vi "Measurement Logic.vi"() -> ()   [LabVIEW 2021, in "Short-Circuit.lvlib"]
uses:
  Short-Circuit.lvlib
  <vilib>/Plug-In SDKs/Measurements/Measure Call Context/Measure Call Context.lvclass
  Measurement Configuration.ctl
  Measurement Results.ctl
  Controls/LED_SCT_Data.ctl
  <instrlib>/niDCPower/nidcpower.llb/niDCPower Source Mode.ctl
  <instrlib>/niDCPower/nidcpower.llb/niDCPower Wait For Event - Event.ctl
  <instrlib>/niSwitch/niSwitch.llb/niSwitch Relay Action.ctl
  <instrlib>/niDMM/nidmm.llb/niDMM Function.ctl
  <instrlib>/niDCPower/nidcpower.llb/niDCPower Output Function.ctl
  <instrlib>/niDCPower/nidcpower.llb/niDCPower Get Channel Name From String.vi
  <instrlib>/niDMM/nidmm.llb/niDMM Configure Measurement Digits.vi
  <instrlib>/niDCPower/nidcpower.llb/niDCPower Configure Digital Edge Source Trigger With Channels.vi
  <instrlib>/niDCPower/nidcpower.llb/niDCPower Configure Digital Edge Measure Trigger With Channels.vi
panel:
  out "measurement results":T1={"Status"="Empty", "Source voltages"=[0.0], "Load voltages"=[0.0], "Source Current"=[0.0], "Load Current"=[0.0]}
  in  "measurement configuration":T2={"DUT setup time"=0.5, "Source delay"=0.5, "Aperture time"=0.5, "Source resource name"="Lorem ipsum dolor sit", "Source sense"=64, "Source current limit"=2.0, "Source maximum power"=20.0, "Source Voltage (Vo)"=3.5, "Load resource name"="", "Load sense"=-64, "Load voltage limit range"=60.0, "Load Voltage Limit"=6.0, "Load Current Level (Io)"=0.1, "Switch resource name"="", "Switch - Load Relay Name"="", "Switch - DMM Relay Name"="", "Relay Topology"="Configured Topology", "DMM resource name"="", "DMM Current Range(A)"=3.0, "SC - Trigger Delay (sec)"=5.0, "SC - Hold Delay (sec)"=5.0, "Resolution in Digits"=6.5} {"Resolution in Digits" items=["3 1/2"=3.5, "4 1/2"=4.5, "5 1/2"=5.5, "6 1/2"=6.5, "7 1/2"=7.5]; "Load Current Level (Io)" format="%.3f"; "Source Voltage (Vo)" format="%.2f"; "Load sense" items=["Local"=1008, "Remote"=1009]; "Source sense" items=["Local"=1008, "Remote"=1009]; "Aperture time" format="%#_6p"; "Source delay" format="%#_6p"; "DUT setup time" format="%#_6p"}
  out "measure call context out":refnum<class "Measure Call Context.lvclass">
  in  "measure call context in":refnum<class "Measure Call Context.lvclass">
  out "error out":errorcluster
  in  "error in":errorcluster
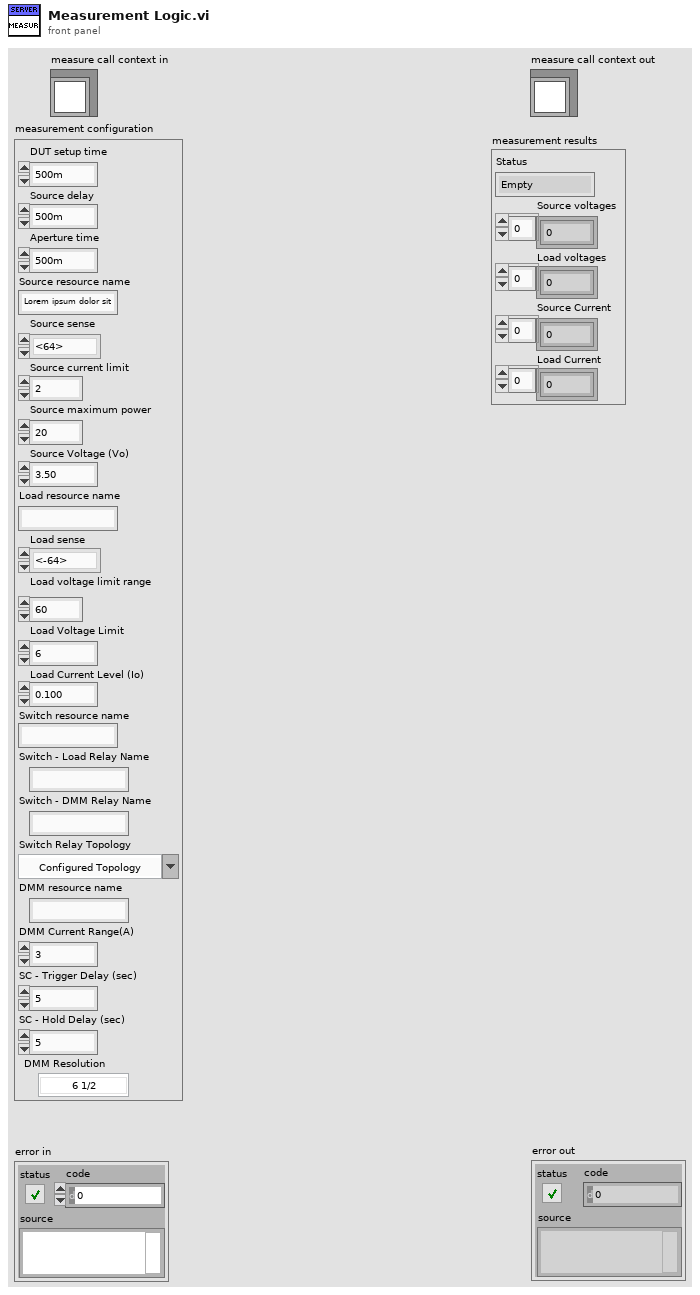
[diagram p1: front panel]
types:
  T1 = typedef "Short-Circuit.lvlib/Measurement Results.ctl" = cluster{"Status":string, "Source voltages":dbl[], "Load voltages":dbl[], "Source Current":dbl[], "Load Current":dbl[]}
  T2 = typedef "Short-Circuit.lvlib/Measurement Configuration.ctl" = cluster{"DUT setup time":dbl, "Source delay":dbl, "Aperture time":dbl, "Source resource name":string, "Source sense":i32, "Source current limit":dbl, "Source maximum power":dbl, "Source Voltage (Vo)":dbl, "Load resource name":string, "Load sense":i32, "Load voltage limit range":dbl, "Load Voltage Limit":dbl, "Load Current Level (Io)":dbl, "Switch resource name":string, "Switch - Load Relay Name":string, "Switch - DMM Relay Name":string, "Relay Topology":string, "DMM resource name":string, "DMM Current Range(A)":dbl, "SC - Trigger Delay (sec)":dbl, "SC - Hold Delay (sec)":dbl, "Resolution in Digits":dbl}
  T3 = typedef "Short-Circuit.lvlib/LED_SCT_Data.ctl" = cluster{"Load channel name":string, "Load out":refnum<k15>, "Source out":refnum<k15>, "Source channel name":string, "Source sequence name":string, "Source terminal name":string, "Measure terminal name":string, "Load Voltage-out":dbl[], "Load Current - out":dbl[], "Source Voltage-out":dbl[], "Source Current - out":dbl[], "Load Relay name":string, "DMM Relay name":string, "Switch out":refnum<k15>, "DMM out":refnum<k15>, "measurement results":T1, "SCT Completed?":bool, "DMM Current Reading":dbl}
  T4 = typedef "niDMM Function.ctl" = enum16{"DC Volts", "AC Volts", "DC Current", "AC Current", "2-wire Resistance", "4-wire Resistance", "Diode", "Frequency", "Period", "AC Volts DC Coupled", "Capacitance", "Inductance", "Temperature"}
  T5 = typedef "niDCPower Wait For Event - Event.ctl" = i32
  T6 = typedef "niDCPower Source Mode.ctl" = i32
  T7 = typedef "niSwitch Relay Action.ctl" = i32
  T8 = typedef "niDCPower Output Function.ctl" = i32
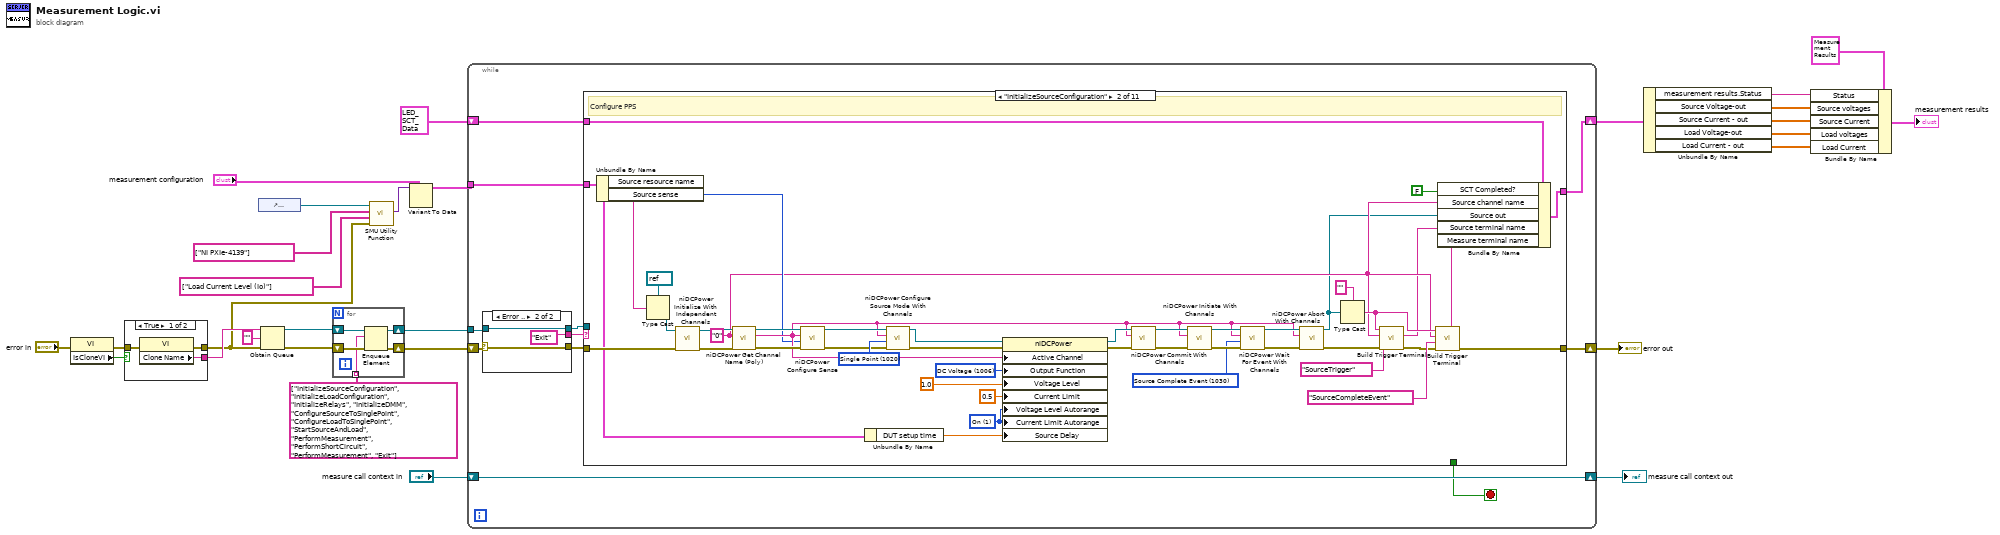
[diagram p0: block diagram]
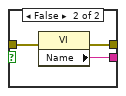
[diagram p2: hidden frame]
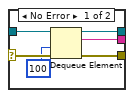
[diagram p3: hidden frame]
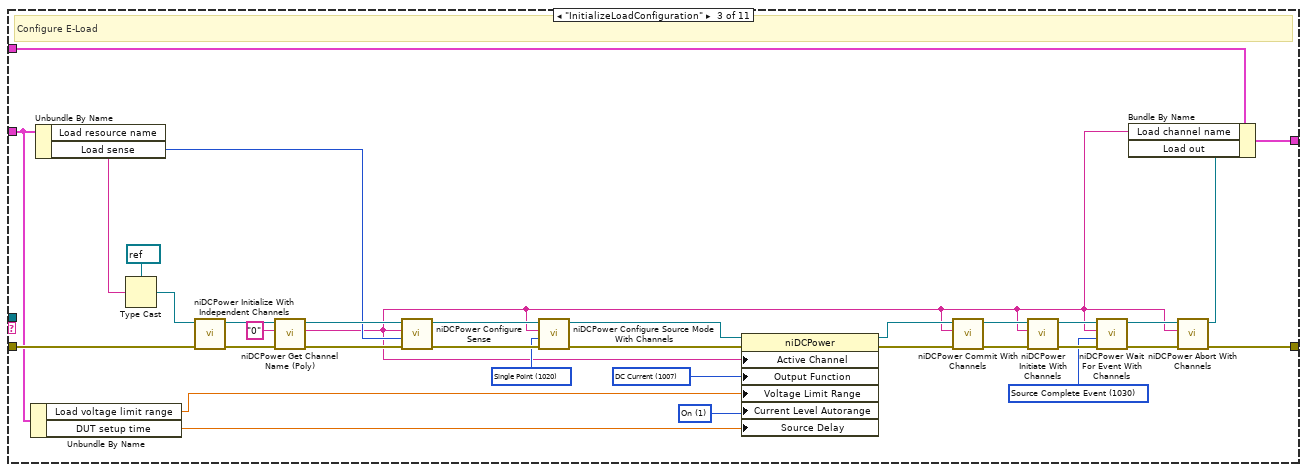
[diagram p5: hidden frame]
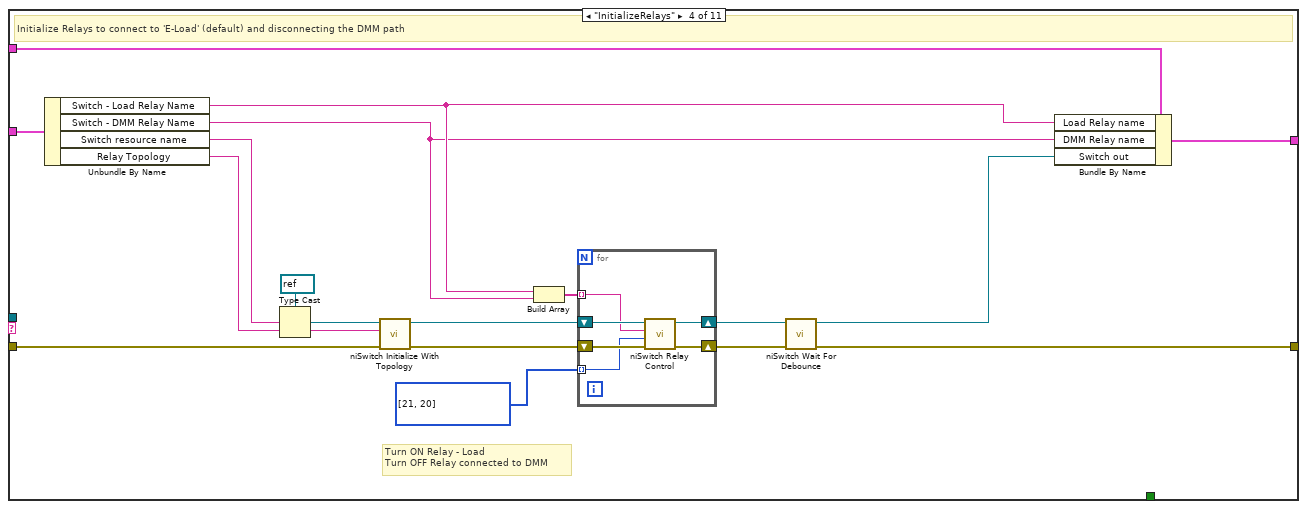
[diagram p6: hidden frame]
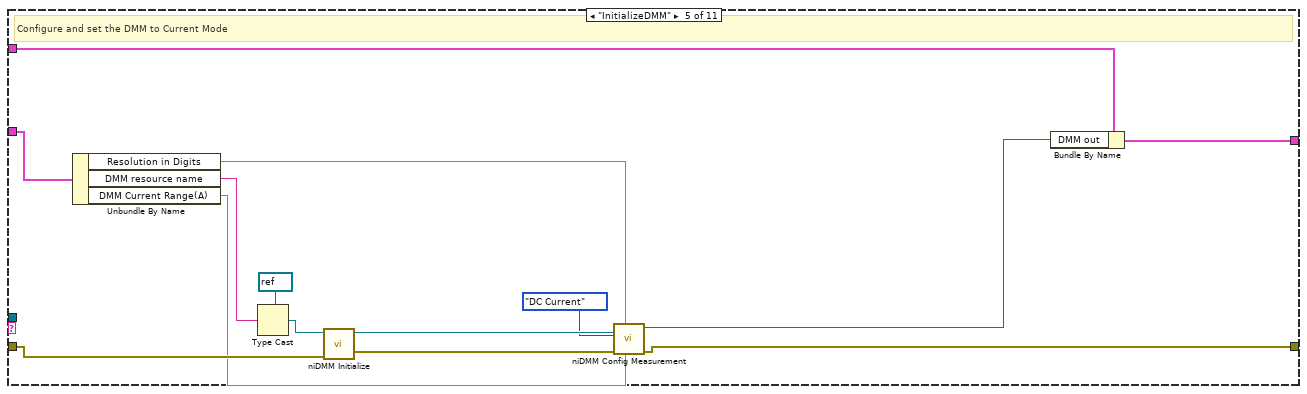
[diagram p7: hidden frame]
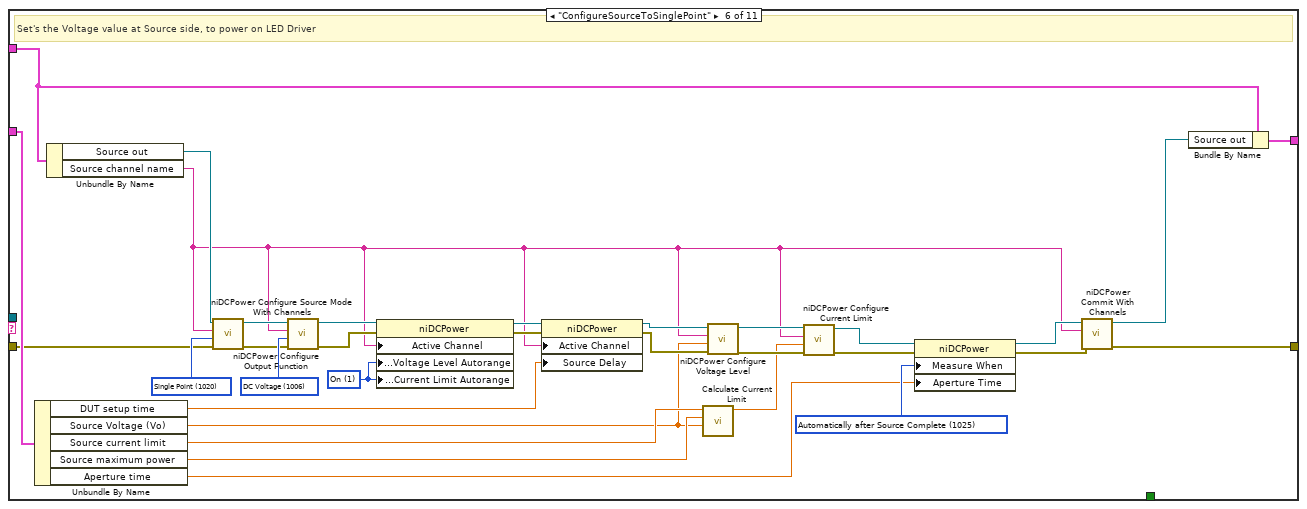
[diagram p8: hidden frame]
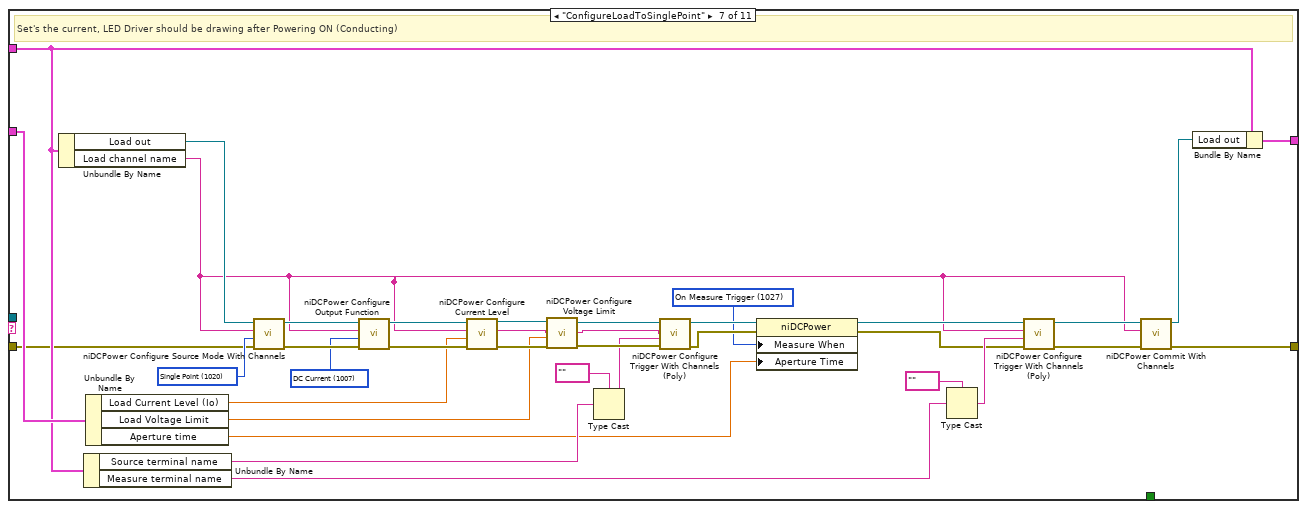
[diagram p9: hidden frame]
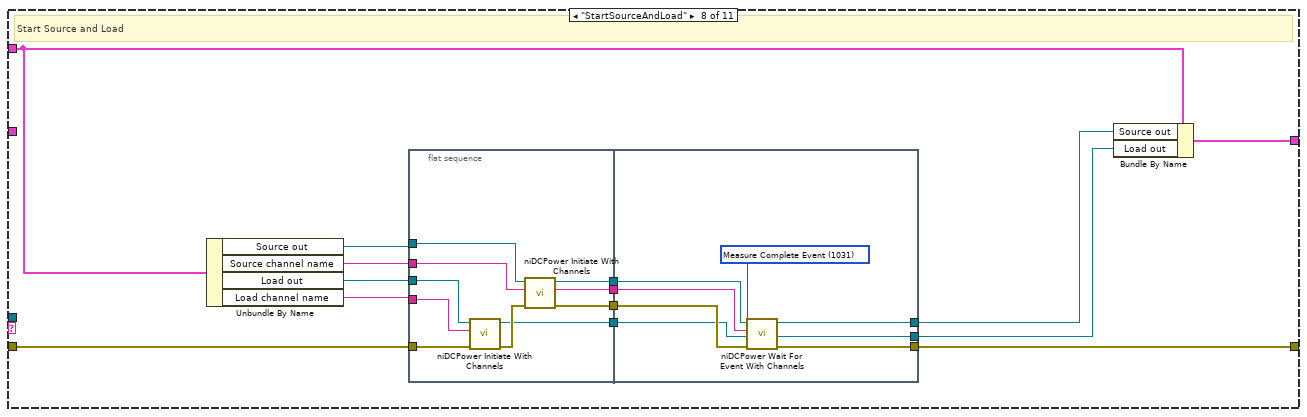
[diagram p10: hidden frame]
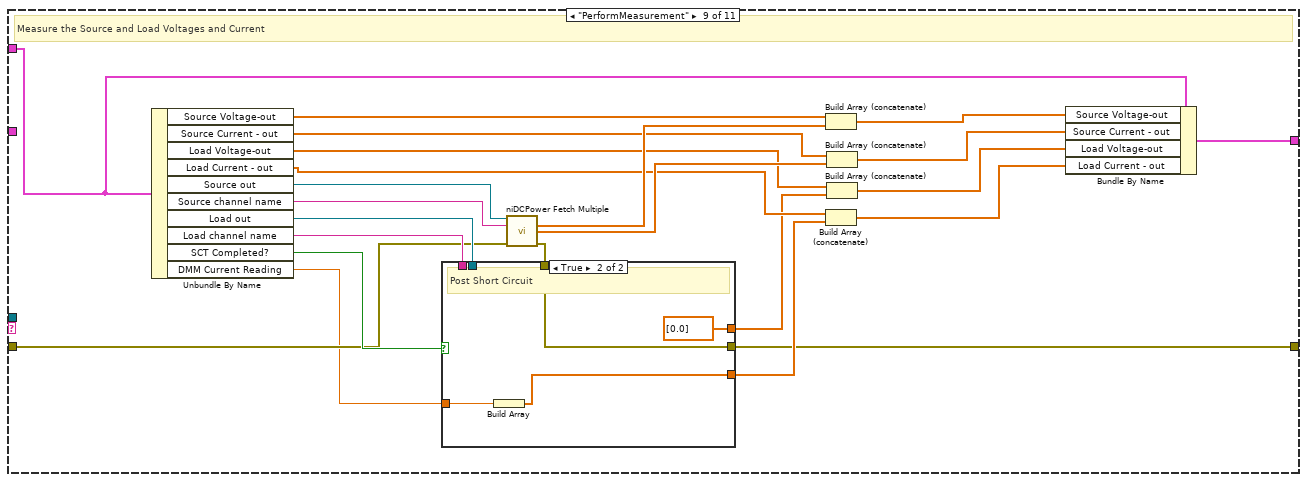
[diagram p11: hidden frame]
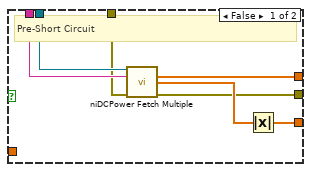
[diagram p12: hidden frame]
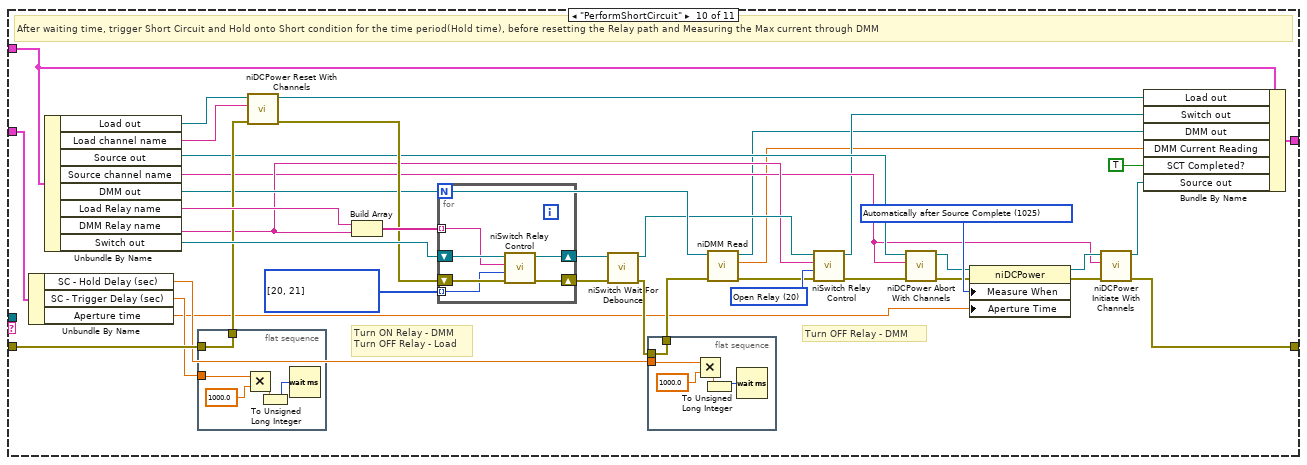
[diagram p13: hidden frame]
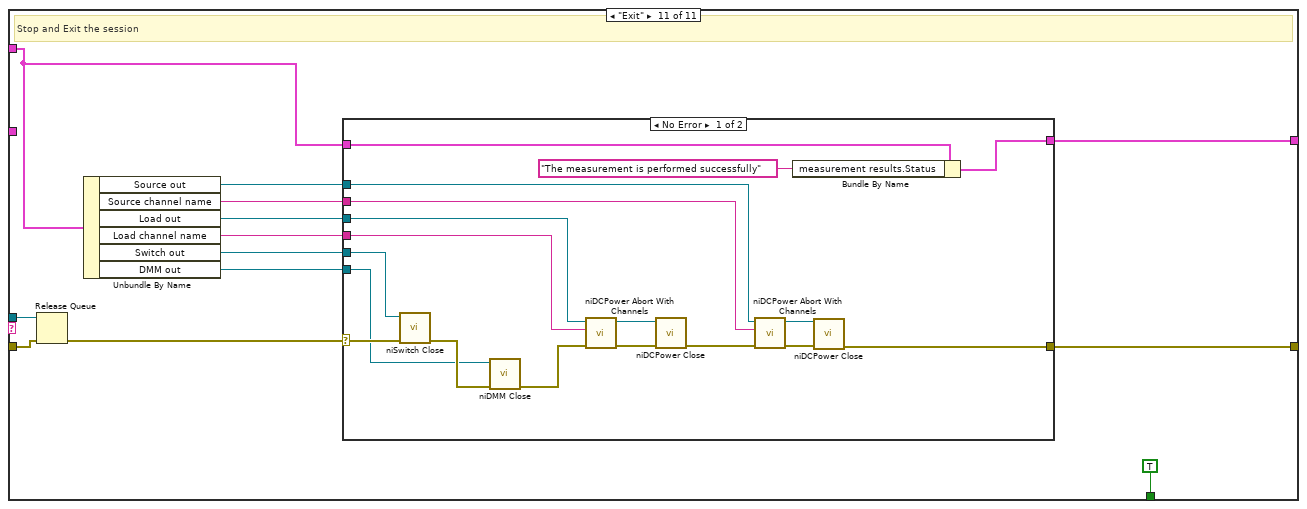
[diagram p14: hidden frame]
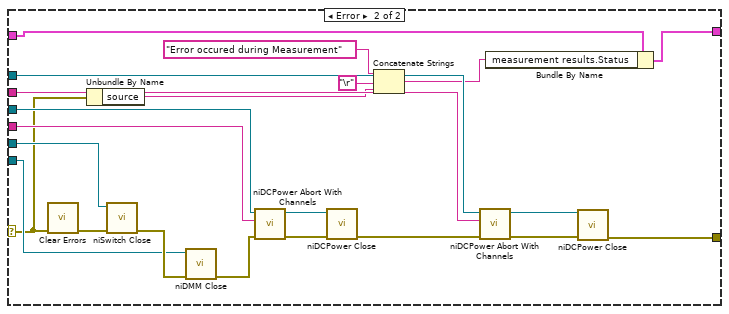
[diagram p15: hidden frame]
diagram:
  n1 = property class="VI"(error in="error in") -> (error out=w28:errorcluster, "IsCloneVI"=w29:bool)  [unwired: 1 in, 1 out]
  n2 = case shown="True" w29 {
    tunnel: [w32 w35] -> w4
    tunnel: [w31 w34] -> w23
    tunnel: w28 -> [w30 w33]
    frame True {
      n3 = property class="VI"(error in=w30) -> (error out=w32:errorcluster, "Clone Name"=w31:string)  [unwired: 1 in, 1 out]
    }
    frame False {
      n4 = property class="VI"(error in=w33) -> (error out=w35:errorcluster, "Name"=w34:string)  [unwired: 1 in, 1 out]
    }
  }
  n5 = control-ref of="measurement configuration"() -> (w7:refnum<vi>)
  n6 = Obtain Queue(name (unnamed)=w23, element data type="", error in (no error)=w4) -> (queue out=w26:refnum<queue>, error out=w27:errorcluster)  [unwired: 2 in, 1 out]
  n7 = for {
    shift-right: [w38] -> w21
    shift-left: w26 -> [w40]
    shift-right: [w37] -> w22
    shift-left: w27 -> [w39]
    tunnel: string[] ["InitializeSourceConfiguration", "InitializeLoadConfiguration", "InitializeRelays", "InitializeDMM", "ConfigureSourceToSinglePoint", "ConfigureLoadToSinglePoint", "StartSourceAndLoad", "PerformMeasurement", "PerformShortCircuit", "PerformMeasurement", "Exit"] ("Step sequence") -> [w36] mode=indexing
    n8 = Enqueue Element(queue=w40, element=w36, error in (no error)=w39) -> (queue out=w38:refnum<queue>, error out=w37:errorcluster)  [unwired: 1 in, 1 out]
  }
  n9 = call "SMU Utility Function.vi"("error in"=w4, "Load Current Parameters"=string[] ["Load Current Level (Io)"], "SMU Model"=string[] ["NI PXIe-4139"], "Measurement Configuration Ref"=w7) -> ("Measurement Configuration Out"=w3:variant)  [unwired: 6 in, 1 out]
  n10 = Variant To Data(type="measurement configuration", Variant=w3) -> (data=w1:T2)  [unwired: 1 in, 1 out]
  n11 = while {
    tunnel: w21 -> [w51]
    shift-right: [w44] -> w16
    shift-left: w22 -> [w50]
    tunnel: w1 -> [w47]
    shift-right: [w45] -> w15
    shift-left: T3 {"Load channel name"="", "Load out"="", "Source out"="", "Source channel name"="", "Source sequence name"="", "Source terminal name"="", "Measure terminal name"="", "Load Voltage-out"=[], "Load Current - out"=[], "Source Voltage-out"=[], "Source Current - out"=[], "Load Relay name"="", "DMM Relay name"="", "Switch out"="", "DMM out"="", "measurement results"={"Status"="Empty", "Source voltages"=[0.0], "Load voltages"=[0.0], "Source Current"=[0.0], "Load Current"=[0.0]}, "SCT Completed?"=FALSE, "DMM Current Reading"=0.0} ("Cluster") -> [w46]
    shift-right: [w43] -> w17
    shift-left: "measure call context in" -> [w43]
    stop <- w41 stop-if-true
    n12 = case shown="Error .." w50 {
      selector: w50 -> [w55 w59]
      tunnel: w51 -> [w57 w58]
      tunnel: [w56 "Exit" ("t")] -> w48
      tunnel: [w54 w59] -> w49
      tunnel: [w52 w58] -> w42
      frame No Error {
        n13 = Dequeue Element(queue=w57, timeout in ms (-1)=100, error in (no error)=w55) -> (queue out=w52:refnum<queue>, element=w56:string, error out=w54:errorcluster)  [unwired: 1 out]
      }
      frame Error {
      }
    }
    n14 = case shown="\"InitializeSourceConfiguration\"" w48 {
      tunnel: w49 -> [w62 w83 w116 w141 w171 w179 w211 w250 w278 w336 w375]
      tunnel: w47 -> [_ w78 w114 w152 w175 w186 w221 _ _ w337 _]
      tunnel: w46 -> [w61 w72 w112 w147 w168 w191 w215 w249 w284 w345 w373]
      tunnel: [w61 w67 w109 w143 w166 w189 w212 w246 w279 w310 w368] -> w45
      tunnel: [w62 w64 w110 w142 w165 w188 w213 w245 w276 w315 w367] -> w44
      tunnel: w42 -> [_ _ _ _ _ _ _ _ _ _ w376]
      tunnel: [_ _ _ _ _ _ _ _ _ _ TRUE] -> w41
      frame "", Default {
      }
      frame "InitializeSourceConfiguration" {
        w71 = "0" ("index")
        w90 = 1 items=["Off", "On"] ("Source:DC Voltage:Voltage Level Autorange")
        w91 = T5 1030 items=["Source Complete Event"=1030, "Measure Complete Event"=1031, "Sequence Iteration Complete Event"=1032, "Sequence Engine Done Event"=1033, "Pulse Complete Event"=1051, "Ready For Pulse Trigger Event"=1052] ("event")
        w102 = T6 1020 items=["Single Point"=1020, "Sequence"=1021] ("source mode")
        w97 = 1006 items=["DC Voltage"=1006, "DC Current"=1007, "Pulse Voltage"=1049, "Pulse Current"=1050] ("Source:Output Function")
        # "Configure PPS"
        n15 = Unbundle By Name(w78) -> ("Source resource name"=w81:string, "Source sense"=w79:i32)
        n16 = Type Cast(type=refnum<k15> refnum ("resource name"), x=w81) -> (*(type *) &x=w80:refnum<k15>)
        n17 = call <instrlib>:"niDCPower Initialize With Independent Channels.vi"("error in (no error)"=w83, "resource name"=w80) -> ("error out"=w88:errorcluster, "instrument handle out"=w92:refnum<k15>)  [unwired: 8 in]
        n18 = call-poly <instrlib>:"niDCPower Get Channel Name (Poly).vi"("error in (no error)"=w88, "index"=w71, "instrument handle"=w92) -> ("error out"=w87:errorcluster, "name"=w84:string, "instrument handle out"=w89:refnum<k15>)  [unwired: 6 in]
        n19 = call <instrlib>:"niDCPower Configure Sense.vi"("error in (no error)"=w87, "sense"=w79, "channel name"=w84, "instrument handle"=w89) -> ("error out"=w100:errorcluster, "instrument handle out"=w98:refnum<k15>)  [unwired: 6 in]
        n20 = Unbundle By Name(w78) -> ("DUT setup time"=w77:dbl)
        n21 = call <instrlib>:"niDCPower Configure Source Mode With Channels.vi"("error in (no error)"=w100, "source mode"=w102, "channel name"=w84, "instrument handle"=w98) -> ("error out"=w101:errorcluster, "instrument handle out"=w99:refnum<k15>)  [unwired: 6 in]
        n22 = property class="niDCPower"(reference=w99, error in=w101, "Active Channel"=w84, "Output Function"=w97, "Voltage Level"=1.0 ("Source:DC Voltage:Voltage Level"), "Current Limit"=0.5 ("Source:DC Voltage:Current Limit"), "Voltage Level Autorange"=w90, "Current Limit Autorange"=w90, "Source Delay"=w77) -> (reference out=w103:refnum<k15>, error out=w104:errorcluster)
        n23 = call <instrlib>:"niDCPower Commit With Channels.vi"("error in (no error)"=w104, "channel name"=w84, "instrument handle"=w103) -> ("error out"=w106:errorcluster, "instrument handle out"=w105:refnum<k15>)  [unwired: 7 in]
        n24 = call <instrlib>:"niDCPower Initiate With Channels.vi"("error in (no error)"=w106, "channel name"=w84, "instrument handle"=w105) -> ("error out"=w93:errorcluster, "instrument handle out"=w94:refnum<k15>)  [unwired: 7 in]
        n25 = call <instrlib>:"niDCPower Wait For Event With Channels.vi"("error in (no error)"=w93, "event"=w91, "channel name"=w84, "instrument handle"=w94) -> ("error out"=w96:errorcluster, "instrument handle out"=w95:refnum<k15>)  [unwired: 6 in]
        n26 = call <instrlib>:"niDCPower Abort With Channels.vi"("error in (no error)"=w96, "channel name"=w84, "instrument handle"=w95) -> ("error out"=w66:errorcluster, "instrument handle out"=w70:refnum<k15>)  [unwired: 7 in]
        n27 = Type Cast(type="", x=w70) -> (*(type *) &x=w75:string)
        n28 = call "Build Trigger Terminal.vi"("error in (no error)"=w66, "Trigger/Event Name"="SourceTrigger", "Channel Name"=w71, "Resource Name"=w75) -> ("error out"=w65:errorcluster, "Terminal Name"=w69:string)  [unwired: 6 in]
        n29 = call "Build Trigger Terminal.vi"("error in (no error)"=w65, "Trigger/Event Name"="SourceCompleteEvent", "Channel Name"=w71, "Resource Name"=w75) -> ("error out"=w64:errorcluster, "Terminal Name"=w68:string)  [unwired: 6 in]
        n30 = Bundle By Name(cluster=w72, "SCT Completed?"=FALSE, "Source channel name"=w71, "Source out"=w70, "Source terminal name"=w69, "Measure terminal name"=w68) -> (w67:T3)
      }
      frame "InitializeLoadConfiguration" {
        w121 = T6 1020 items=["Single Point"=1020, "Sequence"=1021] ("source mode")
        w122 = T5 1030 items=["Source Complete Event"=1030, "Measure Complete Event"=1031, "Sequence Iteration Complete Event"=1032, "Sequence Engine Done Event"=1033, "Pulse Complete Event"=1051, "Ready For Pulse Trigger Event"=1052] ("event")
        w123 = 1 items=["Off", "On"] ("Source:DC Current:Current Level Autorange")
        w124 = 1007 items=["DC Voltage"=1006, "DC Current"=1007, "Pulse Voltage"=1049, "Pulse Current"=1050] ("Source:Output Function")
        # "Configure E-Load"
        n31 = Unbundle By Name(w114) -> ("Load voltage limit range"=w108:dbl, "DUT setup time"=w113:dbl)
        n32 = Unbundle By Name(w114) -> ("Load resource name"=w118:string, "Load sense"=w115:i32)
        n33 = Type Cast(type=refnum<k15> refnum ("resource name"), x=w118) -> (*(type *) &x=w117:refnum<k15>)
        n34 = call <instrlib>:"niDCPower Initialize With Independent Channels.vi"("error in (no error)"=w116, "resource name"=w117) -> ("error out"=w139:errorcluster, "instrument handle out"=w137:refnum<k15>)  [unwired: 8 in]
        n35 = call-poly <instrlib>:"niDCPower Get Channel Name (Poly).vi"("error in (no error)"=w139, "index"="0", "instrument handle"=w137) -> ("error out"=w140:errorcluster, "name"=w111:string, "instrument handle out"=w138:refnum<k15>)  [unwired: 6 in]
        n36 = call <instrlib>:"niDCPower Configure Sense.vi"("error in (no error)"=w140, "sense"=w115, "channel name"=w111, "instrument handle"=w138) -> ("error out"=w131:errorcluster, "instrument handle out"=w132:refnum<k15>)  [unwired: 6 in]
        n37 = call <instrlib>:"niDCPower Configure Source Mode With Channels.vi"("error in (no error)"=w131, "source mode"=w121, "channel name"=w111, "instrument handle"=w132) -> ("error out"=w129:errorcluster, "instrument handle out"=w130:refnum<k15>)  [unwired: 6 in]
        n38 = property class="niDCPower"(reference=w130, error in=w129, "Active Channel"=w111, "Output Function"=w124, "Voltage Limit Range"=w108, "Current Level Autorange"=w123, "Source Delay"=w113) -> (reference out=w128:refnum<k15>, error out=w127:errorcluster)
        n39 = call <instrlib>:"niDCPower Commit With Channels.vi"("error in (no error)"=w127, "channel name"=w111, "instrument handle"=w128) -> ("error out"=w126:errorcluster, "instrument handle out"=w125:refnum<k15>)  [unwired: 7 in]
        n40 = call <instrlib>:"niDCPower Initiate With Channels.vi"("error in (no error)"=w126, "channel name"=w111, "instrument handle"=w125) -> ("error out"=w136:errorcluster, "instrument handle out"=w135:refnum<k15>)  [unwired: 7 in]
        n41 = call <instrlib>:"niDCPower Wait For Event With Channels.vi"("error in (no error)"=w136, "event"=w122, "channel name"=w111, "instrument handle"=w135) -> ("error out"=w133:errorcluster, "instrument handle out"=w134:refnum<k15>)  [unwired: 6 in]
        n42 = call <instrlib>:"niDCPower Abort With Channels.vi"("error in (no error)"=w133, "channel name"=w111, "instrument handle"=w134) -> ("error out"=w110:errorcluster, "instrument handle out"=w107:refnum<k15>)  [unwired: 7 in]
        n43 = Bundle By Name(cluster=w112, "Load channel name"=w111, "Load out"=w107) -> (w109:T3)
      }
      frame "InitializeRelays" {
        w155 = T7[] [21, 20] items=["Open Relay"=20, "Close Relay"=21]
        # "Turn ON Relay - Load\nTurn OFF Relay connected to DMM"
        # "Initialize Relays to connect to 'E-Load' (default) and disconnecting the DMM path"
        n44 = Unbundle By Name(w152) -> ("Switch - Load Relay Name"=w145:string, "Switch - DMM Relay Name"=w144:string, "Switch resource name"=w150:string, "Relay Topology"=w148:string)
        n45 = Type Cast(type=refnum<k15> refnum ("resource name"), x=w150) -> (*(type *) &x=w149:refnum<k15>)
        n46 = call <instrlib>:"niSwitch Initialize With Topology.vi"("error in (no error)"=w141, "topology name"=w148, "resource name"=w149) -> ("error out"=w157:errorcluster, "instrument handle out"=w158:refnum<k15>)  [unwired: 2 in, 5 out]
        n47 = Build Array(w145, w144) -> (w156:string[])
        n48 = for {
          tunnel: w156 -> [w162] mode=indexing
          tunnel: w155 -> [w161] mode=indexing
          shift-right: [w159] -> w153
          shift-left: w157 -> [w163]
          shift-right: [w160] -> w154
          shift-left: w158 -> [w164]
          n49 = call <instrlib>:"niSwitch Relay Control.vi"("error in (no error)"=w163, "relay action (Close Relay)"=w161, "relay names"=w162, "instrument handle"=w164) -> ("error out"=w159:errorcluster, "instrument handle out"=w160:refnum<k15>)  [unwired: 6 out]
        }
        n50 = call <instrlib>:"niSwitch Wait For Debounce.vi"("error in (no error)"=w153, "instrument handle"=w154) -> ("error out"=w142:errorcluster, "instrument handle out"=w146:refnum<k15>)  [unwired: 1 in, 7 out]
        n51 = Bundle By Name(cluster=w147, "Load Relay name"=w145, "DMM Relay name"=w144, "Switch out"=w146) -> (w143:T3)
      }
      frame "InitializeDMM" {
        # "Configure and set the DMM to Current Mode"
        n52 = Unbundle By Name(w175) -> ("Resolution in Digits"=w170:dbl, "DMM resource name"=w173:string, "DMM Current Range(A)"=w169:dbl)
        n53 = Type Cast(type=refnum<k15> refnum ("resource name"), x=w173) -> (*(type *) &x=w172:refnum<k15>)
        n54 = call <instrlib>:"niDMM Initialize.vi"("error in (no error)"=w171, "Instrument Descriptor"=w172) -> ("error out"=w176:errorcluster, "instrument handle out"=w178:refnum<k15>)  [unwired: 8 in]
        n55 = call-poly <instrlib>:"niDMM Config Measurement.vi"("Range"=w169, "Resolution in Digits"=w170, "error in (no error)"=w176, "Function"=niDMM_Function."DC Current", "instrument handle"=w178) -> ("error out"=w165:errorcluster, "instrument handle out"=w167:refnum<k15>)  [unwired: 5 in]
        n56 = Bundle By Name(cluster=w168, "DMM out"=w167) -> (w166:T3)
      }
      frame "ConfigureSourceToSinglePoint" {
        w201 = 1025 items=["Automatically after Source Complete"=1025, "On Demand"=1026, "On Measure Trigger"=1027] ("Measurement:Advanced:Measure When")
        w206 = 1 items=["Off", "On"] ("DC Voltage:Voltage Level Autorange")
        w205 = T8 1006 items=["DC Voltage"=1006, "DC Current"=1007, "Pulse Voltage"=1049, "Pulse Current"=1050] ("output function")
        w204 = T6 1020 items=["Single Point"=1020, "Sequence"=1021] ("source mode")
        # "Set's the Voltage value at Source side, to power on LED Driver"
        n57 = Unbundle By Name(w186) -> ("DUT setup time"=w185:dbl, "Source Voltage (Vo)"=w182:dbl, "Source current limit"=w184:dbl, "Source maximum power"=w183:dbl, "Aperture time"=w180:dbl)
        n58 = Unbundle By Name(w191) -> ("Source out"=w192:refnum<k15>, "Source channel name"=w187:string)
        n59 = call <instrlib>:"niDCPower Configure Source Mode With Channels.vi"("error in (no error)"=w179, "source mode"=w204, "channel name"=w187, "instrument handle"=w192) -> ("error out"=w202:errorcluster, "instrument handle out"=w203:refnum<k15>)  [unwired: 6 in]
        n60 = call <instrlib>:"niDCPower Configure Output Function.vi"("error in (no error)"=w202, "output function"=w205, "channel name"=w187, "instrument handle"=w203) -> ("error out"=w210:errorcluster, "instrument handle out"=w209:refnum<k15>)  [unwired: 6 out]
        n61 = property class="niDCPower"(reference=w209, error in=w210, "Active Channel"=w187, "Source:DC Voltage:Voltage Level Autorange"=w206, "Source:DC Voltage:Current Limit Autorange"=w206) -> (reference out=w207:refnum<k15>, error out=w208:errorcluster)
        n62 = property class="niDCPower"(reference=w207, error in=w208, "Active Channel"=w187, "Source Delay"=w185) -> (reference out=w198:refnum<k15>, error out=w197:errorcluster)
        n63 = call "Calculate Current Limit.vi"("Voltage value"=w182, "Maximum power"=w183, "Current limit in"=w184) -> ("Current limit out"=w181:dbl)  [unwired: 8 in]
        n64 = call <instrlib>:"niDCPower Configure Voltage Level.vi"("error in (no error)"=w197, "voltage level"=w182, "channel name"=w187, "instrument handle"=w198) -> ("error out"=w195:errorcluster, "instrument handle out"=w196:refnum<k15>)  [unwired: 6 in]
        n65 = call <instrlib>:"niDCPower Configure Current Limit.vi"("error in (no error)"=w195, "current limit"=w181, "channel name"=w187, "instrument handle"=w196) -> ("error out"=w193:errorcluster, "instrument handle out"=w194:refnum<k15>)  [unwired: 6 in]
        n66 = property class="niDCPower"(reference=w194, error in=w193, "Measure When"=w201, "Aperture Time"=w180) -> (reference out=w199:refnum<k15>, error out=w200:errorcluster)
        n67 = call <instrlib>:"niDCPower Commit With Channels.vi"("error in (no error)"=w200, "channel name"=w187, "instrument handle"=w199) -> ("error out"=w188:errorcluster, "instrument handle out"=w190:refnum<k15>)  [unwired: 7 in]
        n68 = Bundle By Name(cluster=w191, "Source out"=w190) -> (w189:T3)
      }
      frame "ConfigureLoadToSinglePoint" {
        w226 = T8 1007 items=["DC Voltage"=1006, "DC Current"=1007, "Pulse Voltage"=1049, "Pulse Current"=1050] ("output function")
        w228 = 1027 items=["Automatically after Source Complete"=1025, "On Demand"=1026, "On Measure Trigger"=1027] ("Measurement:Advanced:Measure When")
        w227 = T6 1020 items=["Single Point"=1020, "Sequence"=1021] ("source mode")
        # "Set's the current, LED Driver should be drawing after Powering ON (Conducting)"
        n69 = Unbundle By Name(w215) -> ("Load out"=w223:refnum<k15>, "Load channel name"=w222:string)
        n70 = Unbundle By Name(w215) -> ("Source terminal name"=w218:string, "Measure terminal name"=w217:string)
        n71 = Unbundle By Name(w221) -> ("Load Current Level (Io)"=w220:dbl, "Load Voltage Limit"=w219:dbl, "Aperture time"=w216:dbl)
        n72 = call <instrlib>:"niDCPower Configure Source Mode With Channels.vi"("error in (no error)"=w211, "source mode"=w227, "channel name"=w222, "instrument handle"=w223) -> ("error out"=w233:errorcluster, "instrument handle out"=w232:refnum<k15>)  [unwired: 6 in]
        n73 = call <instrlib>:"niDCPower Configure Output Function.vi"("error in (no error)"=w233, "output function"=w226, "channel name"=w222, "instrument handle"=w232) -> ("error out"=w239:errorcluster, "instrument handle out"=w240:refnum<k15>)  [unwired: 6 in]
        n74 = call <instrlib>:"niDCPower Configure Current Level.vi"("error in (no error)"=w239, "current level"=w220, "channel name"=w222, "instrument handle"=w240) -> ("error out"=w241:errorcluster, "instrument handle out"=w244:refnum<k15>)  [unwired: 6 in]
        n75 = call <instrlib>:"niDCPower Configure Voltage Limit.vi"("error in (no error)"=w241, "voltage limit"=w219, "channel name"=w222, "instrument handle"=w244) -> ("error out"=w242:errorcluster, "instrument handle out"=w243:refnum<k15>)  [unwired: 6 in]
        n76 = Type Cast(type=tag "" ("input terminal"), x=w218) -> (*(type *) &x=w237:tag)
        n77 = call-poly <instrlib>:"niDCPower Configure Trigger With Channels (Poly).vi"("error in (no error)"=w242, "input terminal"=w237, "channel name"=w222, "instrument handle"=w243) -> ("error out"=w236:errorcluster, "instrument handle out"=w229:refnum<k15>)  [unwired: 6 in]
        n78 = property class="niDCPower"(reference=w229, error in=w236, "Measure When"=w228, "Aperture Time"=w216) -> (reference out=w234:refnum<k15>, error out=w235:errorcluster)
        n79 = Type Cast(type=tag "" ("input terminal"), x=w217) -> (*(type *) &x=w238:tag)
        n80 = call-poly <instrlib>:"niDCPower Configure Trigger With Channels (Poly).vi"("error in (no error)"=w235, "input terminal"=w238, "channel name"=w222, "instrument handle"=w234) -> ("error out"=w231:errorcluster, "instrument handle out"=w230:refnum<k15>)  [unwired: 6 in]
        n81 = call <instrlib>:"niDCPower Commit With Channels.vi"("error in (no error)"=w231, "channel name"=w222, "instrument handle"=w230) -> ("error out"=w213:errorcluster, "instrument handle out"=w214:refnum<k15>)  [unwired: 7 in]
        n82 = Bundle By Name(cluster=w215, "Load out"=w214) -> (w212:T3)
      }
      frame "StartSourceAndLoad" {
        # "Start Source and Load"
        n83 = Unbundle By Name(w249) -> ("Source out"=w254:refnum<k15>, "Source channel name"=w253:string, "Load out"=w252:refnum<k15>, "Load channel name"=w251:string)
        n84 = flat-sequence {
          tunnel: [w266] -> w258
          tunnel: [w265] -> w257
          tunnel: w250 -> [w264]
          tunnel: w252 -> [w263]
          tunnel: w254 -> [w262]
          tunnel: w253 -> [w260]
          tunnel: w251 -> [w259]
          tunnel: [w261] -> w256
          tunnel: [w260] -> w255
          tunnel: w258 -> [w272]
          tunnel: w257 -> [w269]
          tunnel: [w269] -> w247
          tunnel: w256 -> [w274]
          tunnel: w255 -> [w273]
          tunnel: [w271] -> w245
          tunnel: [w270] -> w248
          frame #0 {
            n85 = call <instrlib>:"niDCPower Initiate With Channels.vi"("error in (no error)"=w264, "channel name"=w259, "instrument handle"=w263) -> ("error out"=w267:errorcluster, "instrument handle out"=w265:refnum<k15>)  [unwired: 7 in]
            n86 = call <instrlib>:"niDCPower Initiate With Channels.vi"("error in (no error)"=w267, "channel name"=w260, "instrument handle"=w262) -> ("error out"=w266:errorcluster, "instrument handle out"=w261:refnum<k15>)  [unwired: 7 in]
          }
          frame #1 {
            w268 = T5 1031 items=["Source Complete Event"=1030, "Measure Complete Event"=1031, "Sequence Iteration Complete Event"=1032, "Sequence Engine Done Event"=1033, "Pulse Complete Event"=1051, "Ready For Pulse Trigger Event"=1052] ("event")
            n87 = call <instrlib>:"niDCPower Wait For Event With Channels.vi"("error in (no error)"=w272, "event"=w268, "channel name"=w273, "instrument handle"=w274) -> ("error out"=w271:errorcluster, "instrument handle out"=w270:refnum<k15>)  [unwired: 6 in]
          }
        }
        n88 = Bundle By Name(cluster=w249, "Source out"=w248, "Load out"=w247) -> (w246:T3)
      }
      frame "PerformMeasurement" {
        # "Measure the Source and Load Voltages and Current"
        n89 = Unbundle By Name(w284) -> ("Source Voltage-out"=w292:dbl[], "Source Current - out"=w290:dbl[], "Load Voltage-out"=w288:dbl[], "Load Current - out"=w287:dbl[], "Source out"=w297:refnum<k15>, "Source channel name"=w296:string, "Load out"=w295:refnum<k15>, "Load channel name"=w294:string, "SCT Completed?"=w293:bool, "DMM Current Reading"=w275:dbl)
        n90 = call <instrlib>:"niDCPower Fetch Multiple.vi"("instrument handle"=w297, "channel name"=w296, "error in (no error)"=w278) -> ("voltage measurements"=w291:dbl[], "current measurements"=w289:dbl[], "error out"=w277:errorcluster)  [unwired: 2 in, 8 out]
        n91 = case shown="True" w293 {
          tunnel: w295 -> [w304 _]
          tunnel: w294 -> [w303 _]
          tunnel: [w302 dbl[] [0.0] ("voltage measurements")] -> w286
          tunnel: [w298 w306] -> w285
          tunnel: w277 -> [w300 w305]
          tunnel: [w299 w305] -> w276
          tunnel: w275 -> [_ w307]
          frame False {
            # "Pre-Short Circuit"
            n92 = call <instrlib>:"niDCPower Fetch Multiple.vi"("instrument handle"=w304, "channel name"=w303, "error in (no error)"=w300) -> ("voltage measurements"=w302:dbl[], "current measurements"=w301:dbl[], "error out"=w299:errorcluster)  [unwired: 2 in, 8 out]
            n93 = Absolute Value(x=w301) -> (abs(x)=w298:dbl[])
          }
          frame True {
            # "Post Short Circuit"
            n94 = Build Array(w307) -> (w306:dbl[])
          }
        }
        n95 = Build Array (concatenate)(w292, w291) -> (w283:dbl[])
        n96 = Build Array (concatenate)(w287, w285) -> (w280:dbl[])
        n97 = Build Array (concatenate)(w290, w289) -> (w282:dbl[])
        n98 = Build Array (concatenate)(w288, w286) -> (w281:dbl[])
        n99 = Bundle By Name(cluster=w284, "Source Voltage-out"=w283, "Source Current - out"=w282, "Load Voltage-out"=w281, "Load Current - out"=w280) -> (w279:T3)
      }
      frame "PerformShortCircuit" {
        w322 = 1025 items=["Automatically after Source Complete"=1025, "On Demand"=1026, "On Measure Trigger"=1027] ("Measurement:Advanced:Measure When")
        w326 = T7 20 items=["Open Relay"=20, "Close Relay"=21] ("relay action (Close Relay)")
        w343 = T7[] [20, 21] items=["Open Relay"=20, "Close Relay"=21]
        # "Turn OFF Relay - DMM"
        # "Turn ON Relay - DMM\nTurn OFF Relay - Load"
        # "After waiting time, trigger Short Circuit and Hold onto Short condition for the time period(Hold time), before resetting the Relay path and Measuring the Max current through DMM"
        n100 = Unbundle By Name(w337) -> ("SC - Hold Delay (sec)"=w331:dbl, "SC - Trigger Delay (sec)"=w330:dbl, "Aperture time"=w319:dbl)
        n101 = Unbundle By Name(w345) -> ("Load out"=w347:refnum<k15>, "Load channel name"=w346:string, "Source out"=w324:refnum<k15>, "Source channel name"=w317:string, "DMM out"=w329:refnum<k15>, "Load Relay name"=w339:string, "DMM Relay name"=w327:string, "Switch out"=w338:refnum<k15>)
        n102 = flat-sequence {
          tunnel: w330 -> [w357]
          tunnel: [w353] -> w335
          tunnel: w336 -> [w353]
          frame #0 {
            n103 = Multiply(x=w357, y=1000.0) -> (x*y=w355:dbl)
            n104 = To Unsigned Long Integer(number=w355) -> (unsigned 32bit integer=w354:u32)
            n105 = Wait (ms)(milliseconds to wait=w354) -> ()  [unwired: 1 out]
          }
        }
        n106 = call <instrlib>:"niDCPower Reset With Channels.vi"("error in (no error)"=w335, "channel name"=w346, "instrument handle"=w347) -> ("error out"=w334:errorcluster, "instrument handle out"=w344:refnum<k15>)  [unwired: 7 in]
        n107 = Build Array(w339, w327) -> (w342:string[])
        n108 = for {
          tunnel: w342 -> [w361] mode=indexing
          tunnel: w343 -> [w360] mode=indexing
          shift-right: [w358] -> w341
          shift-left: w334 -> [w362]
          shift-right: [w359] -> w340
          shift-left: w338 -> [w363]
          n109 = call <instrlib>:"niSwitch Relay Control.vi"("error in (no error)"=w362, "relay action (Close Relay)"=w360, "relay names"=w361, "instrument handle"=w363) -> ("error out"=w358:errorcluster, "instrument handle out"=w359:refnum<k15>)  [unwired: 6 out]
        }
        n110 = call <instrlib>:"niSwitch Wait For Debounce.vi"("error in (no error)"=w341, "instrument handle"=w340) -> ("error out"=w333:errorcluster, "instrument handle out"=w328:refnum<k15>)  [unwired: 1 in, 7 out]
        n111 = flat-sequence {
          tunnel: w331 -> [w352]
          tunnel: [w348] -> w332
          tunnel: w333 -> [w348]
          frame #0 {
            n112 = Multiply(x=w352, y=1000.0) -> (x*y=w350:dbl)
            n113 = To Unsigned Long Integer(number=w350) -> (unsigned 32bit integer=w349:u32)
            n114 = Wait (ms)(milliseconds to wait=w349) -> ()  [unwired: 1 out]
          }
        }
        n115 = call <instrlib>:"niDMM Read.vi"("error in (no error)"=w332, "instrument handle"=w329) -> ("error out"=w325:errorcluster, "Measurement"=w312:dbl, "instrument handle out"=w313:refnum<k15>)  [unwired: 7 in]
        n116 = call <instrlib>:"niSwitch Relay Control.vi"("error in (no error)"=w325, "relay action (Close Relay)"=w326, "relay names"=w327, "instrument handle"=w328) -> ("error out"=w323:errorcluster, "instrument handle out"=w314:refnum<k15>)  [unwired: 6 out]
        n117 = call <instrlib>:"niDCPower Abort With Channels.vi"("error in (no error)"=w323, "channel name"=w317, "instrument handle"=w324) -> ("error out"=w320:errorcluster, "instrument handle out"=w321:refnum<k15>)  [unwired: 7 in]
        n118 = property class="niDCPower"(reference=w321, error in=w320, "Measure When"=w322, "Aperture Time"=w319) -> (reference out=w318:refnum<k15>, error out=w316:errorcluster)
        n119 = call <instrlib>:"niDCPower Initiate With Channels.vi"("error in (no error)"=w316, "channel name"=w317, "instrument handle"=w318) -> ("error out"=w315:errorcluster, "instrument handle out"=w309:refnum<k15>)  [unwired: 7 in]
        n120 = Bundle By Name(cluster=w345, "Load out"=w344, "Switch out"=w314, "DMM out"=w313, "DMM Current Reading"=w312, "SCT Completed?"=TRUE, "Source out"=w309) -> (w310:T3)
      }
      frame "Exit" {
        # "Stop and Exit the session"
        n121 = Release Queue(queue=w376, error in (no error)=w375) -> (error out=w374:errorcluster)  [unwired: 1 in, 2 out]
        n122 = Unbundle By Name(w373) -> ("Source out"=w372:refnum<k15>, "Source channel name"=w371:string, "Load out"=w370:refnum<k15>, "Load channel name"=w369:string, "Switch out"=w366:refnum<k15>, "DMM out"=w365:refnum<k15>)
        n123 = case shown="No Error" w374 {
          selector: w374 -> [w379 w397]
          tunnel: w370 -> [w390 w413]
          tunnel: w369 -> [w391 w410]
          tunnel: w371 -> [w385 w409]
          tunnel: [w386 w412] -> w367
          tunnel: w372 -> [w387 w411]
          tunnel: w373 -> [w383 w408]
          tunnel: [w382 w407] -> w368
          tunnel: w366 -> [w380 w406]
          tunnel: w365 -> [w378 w403]
          frame No Error {
            n124 = call <instrlib>:"niSwitch Close.vi"("error in (no error)"=w379, "instrument handle"=w380) -> ("error out"=w381:errorcluster)  [unwired: 9 in]
            n125 = call <instrlib>:"niDMM Close.vi"("error in (no error)"=w381, "instrument handle"=w378) -> ("error out"=w377:errorcluster)  [unwired: 9 in]
            n126 = call <instrlib>:"niDCPower Abort With Channels.vi"("error in (no error)"=w377, "channel name"=w391, "instrument handle"=w390) -> ("error out"=w388:errorcluster, "instrument handle out"=w389:refnum<k15>)  [unwired: 7 in]
            n127 = call <instrlib>:"niDCPower Close.vi"("error in (no error)"=w388, "instrument handle"=w389) -> ("error out"=w392:errorcluster)  [unwired: 9 in]
            n128 = call <instrlib>:"niDCPower Abort With Channels.vi"("error in (no error)"=w392, "channel name"=w385, "instrument handle"=w387) -> ("error out"=w394:errorcluster, "instrument handle out"=w393:refnum<k15>)  [unwired: 7 in]
            n129 = Bundle By Name(cluster=w383, "measurement results.Status"="The measurement is performed successfully" ("message")) -> (w382:T3)
            n130 = call <instrlib>:"niDCPower Close.vi"("error in (no error)"=w394, "instrument handle"=w393) -> ("error out"=w386:errorcluster)  [unwired: 9 in]
          }
          frame Error {
            n131 = call <vilib>:"Clear Errors.vi"("error in (no error)"=w397) -> ("error out"=w404:errorcluster)  [unwired: 5 in, 1 out]
            n132 = Unbundle By Name(w397) -> ("source"=w396:string)
            n133 = call <instrlib>:"niSwitch Close.vi"("error in (no error)"=w404, "instrument handle"=w406) -> ("error out"=w405:errorcluster)  [unwired: 9 in]
            n134 = call <instrlib>:"niDMM Close.vi"("error in (no error)"=w405, "instrument handle"=w403) -> ("error out"=w400:errorcluster)  [unwired: 9 in]
            n135 = call <instrlib>:"niDCPower Abort With Channels.vi"("error in (no error)"=w400, "channel name"=w410, "instrument handle"=w413) -> ("error out"=w401:errorcluster, "instrument handle out"=w402:refnum<k15>)  [unwired: 7 in]
            n136 = call <instrlib>:"niDCPower Close.vi"("error in (no error)"=w401, "instrument handle"=w402) -> ("error out"=w414:errorcluster)  [unwired: 9 in]
            n137 = Concatenate Strings("Error occured during Measurement" ("message"), "\r", w396) -> (w395:string)
            n138 = call <instrlib>:"niDCPower Abort With Channels.vi"("error in (no error)"=w414, "channel name"=w409, "instrument handle"=w411) -> ("error out"=w416:errorcluster, "instrument handle out"=w415:refnum<k15>)  [unwired: 7 in]
            n139 = Bundle By Name(cluster=w408, "measurement results.Status"=w395) -> (w407:T3)
            n140 = call <instrlib>:"niDCPower Close.vi"("error in (no error)"=w416, "instrument handle"=w415) -> ("error out"=w412:errorcluster)  [unwired: 9 in]
          }
        }
      }
    }
  }
  "error out" <- w16
  "measure call context out" <- w17
  n141 = Unbundle By Name(w15) -> ("measurement results.Status"=w13:string, "Source Voltage-out"=w12:dbl[], "Source Current - out"=w11:dbl[], "Load Voltage-out"=w10:dbl[], "Load Current - out"=w9:dbl[])
  n142 = Bundle By Name(cluster=T1 {"Status"="Empty", "Source voltages"=[0.0], "Load voltages"=[0.0], "Source Current"=[0.0], "Load Current"=[0.0]} ("measurement results"), "Status"=w13, "Source voltages"=w12, "Source Current"=w11, "Load voltages"=w10, "Load Current"=w9) -> (→"measurement results":T1)
